vi "set_edge_attribute.vi"(7 "attribute-name":string, 8 "error in (no error)":errorcluster, 9 "attribute-value":variant, 10 "edge":refnum<class "Edge.lvclass">, 11 "graph":refnum<class "Graph.lvclass">) -> (0 "error out":errorcluster, 3 "graph-out":refnum<class "Graph.lvclass">)   [LabVIEW 2020, in "graph.lvlib" / "Graph.lvclass"]
uses:
  Graph.lvclass
  Edge/Edge.lvclass
  Graph.lvclass/Graph.ctl
  <vilib>/Utility/miscctls.llb/LVMapReplaceAction.ctl
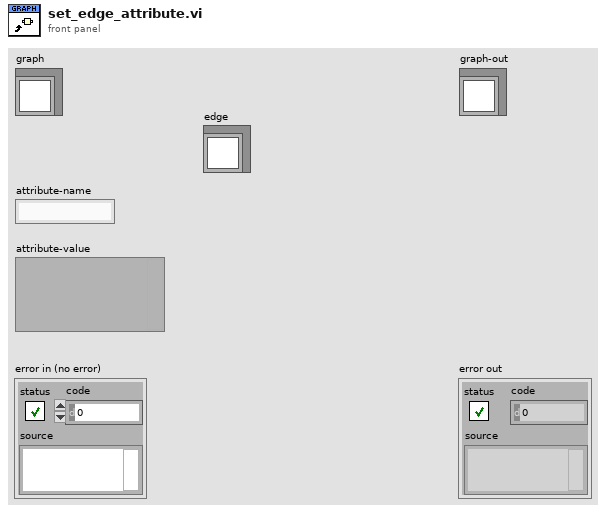
[diagram p1: front panel]
types:
  T1 = typedef "LVMapReplaceAction.ctl" = enum32{"Modify Entry only if found", "Add or Modify Entry", "Delete Entry"}
  T2 = typedef "graph.lvlib/Graph.lvclass/edge-definition-cluster.ctl" = cluster{"source-id":refnum<class "ID.lvclass">, "sink-id":refnum<class "ID.lvclass">}
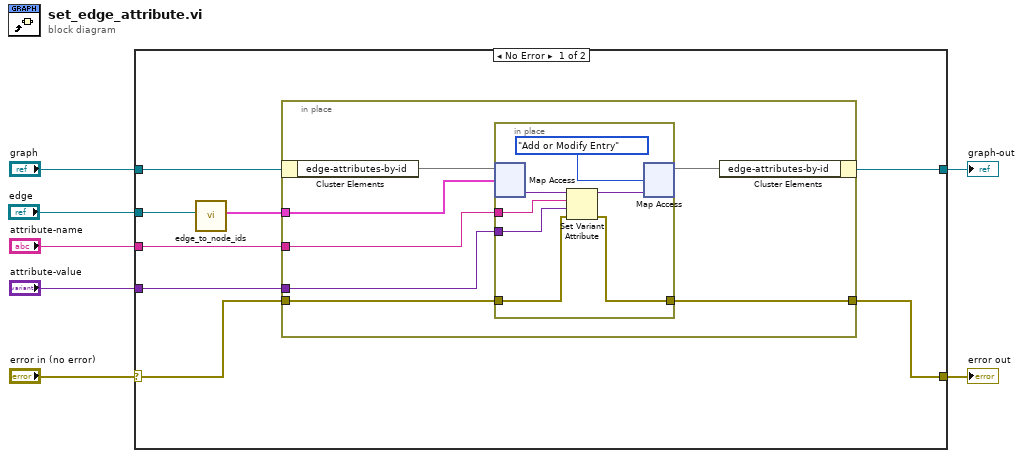
[diagram p0: block diagram]
diagram:
  n1 = case shown="No Error" "error in (no error)" {
    selector: "error in (no error)" -> [w9 w31]
    tunnel: [w8 w31] -> w6
    tunnel: [w13 w30] -> w4
    tunnel: "graph" -> [w12 w30]
    tunnel: "attribute-name" -> [w15 _]
    tunnel: "attribute-value" -> [w14 _]
    tunnel: "edge" -> [w10 _]
    frame No Error {
      n2 = call "edge_to_node_ids.vi"("edge"=w10) -> ("node-ids-cluster"=w11:T2)  [unwired: 10 in]
      n3 = in-place {
        in-place-border: w15 -> [w20]
        in-place-border: w14 -> [w19]
        in-place-border: w11 -> [w18]
        in-place-border: w9 -> [w17]
        in-place-border: [w16] -> w8
        n4 = in-place-cluster #1(w12) -> ("edge-attributes-by-id"=w22:map{T2, variant})
        n5 = in-place {
          in-place-border: w20 -> [w27]
          in-place-border: w19 -> [w26]
          in-place-border: w17 -> [w24]
          in-place-border: [w23] -> w16
          n6 = in-place-map #2(w22, w18) -> (w29:variant)  [unwired: 1 in, 1 out]
          n7 = Set Variant Attribute(Variant=w29, name=w27, value=w26, error in=w24) -> (Variant out=w28:variant, error out=w23:errorcluster)  [unwired: 1 out]
          n8 = in-place-map #2(w28, LVMapReplaceAction."Add or Modify Entry" ("action")) -> (w21:map{T2, variant})  [unwired: 2 out]
        }
        n9 = in-place-cluster #1("edge-attributes-by-id"=w21) -> (w13:refnum<class "Graph.lvclass">)
      }
    }
    frame Error {
    }
  }
  "error out" <- w6
  "graph-out" <- w4
